vi "Create Message Accessor.vi"(8 "error in (no error)":errorcluster, 10 "message name":string, 11 "library in":refnum<vi>) -> (0 "error out":errorcluster, 3 "library out":refnum<vi>)   [LabVIEW 2019, in "gRPC Template Creation Utility.lvlib"]
uses:
  gRPC Template Creation Utility.lvlib
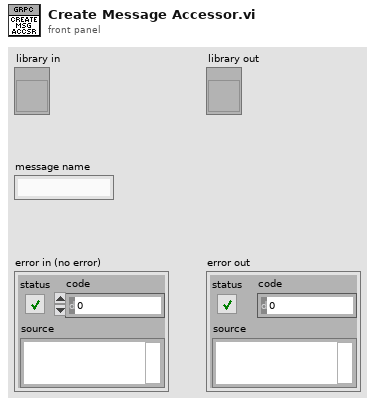
[diagram p1: front panel]
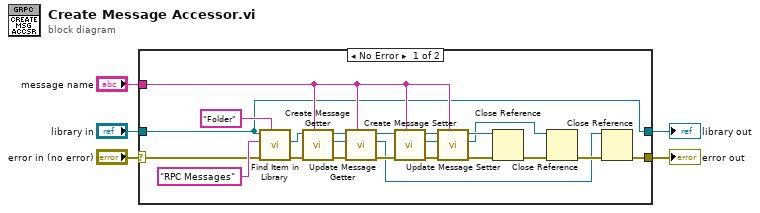
[diagram p0: block diagram]
diagram:
  n1 = case shown="No Error" "error in (no error)" {
    selector: "error in (no error)" -> [w15 w28]
    tunnel: "library in" -> [w14 w29]
    tunnel: "message name" -> [w27 _]
    tunnel: [w16 w28] -> w4
    tunnel: [w14 w29] -> w2
    frame No Error {
      n2 = call "Find Item in Library.vi"("Item Type"="Folder", "error in (no error)"=w15, "Item Name"="RPC Messages", "Library item in"=w14) -> ("error out"=w13:errorcluster, "Project Item (Library Item)"=w21:refnum<vi>)  [unwired: 4 in, 2 out]
      n3 = call "Create Message Getter.vi"("RPC Message Name"=w27, "error in (no error)"=w13, "RPC Messages Folder (ProjectItem) in"=w21) -> ("error out"=w22:errorcluster, "Message Getter out"=w23:refnum<vi>, "RPC Messages Folder (ProjectItem) out"=w24:refnum<vi>)  [unwired: 6 in]
      n4 = call "Update Message Getter.vi"("RPC Message Name"=w27, "error in (no error)"=w22, "Message Getter in"=w23, "RPC Messages Folder (ProjectItem) in"=w24) -> ("error out"=w12:errorcluster, "Message Getter out"=w7:refnum<vi>, "RPC Messages Folder (ProjectItem) out"=w11:refnum<vi>)  [unwired: 5 in]
      n5 = call "Create Message Setter.vi"("RPC Message Name"=w27, "error in (no error)"=w12, "RPC Messages Folder (ProjectItem) in"=w11) -> ("error out"=w20:errorcluster, "Message Setter out"=w18:refnum<vi>, "RPC Messages Folder (ProjectItem) out"=w19:refnum<vi>)  [unwired: 6 in]
      n6 = call "Update Message Setter.vi"("RPC Message Name"=w27, "error in (no error)"=w20, "Message Getter in"=w18, "RPC Messages Folder (ProjectItem) in"=w19) -> ("error out"=w17:errorcluster, "Message Getter out"=w6:refnum<vi>, "RPC Messages Folder (ProjectItem) out"=w8:refnum<vi>)  [unwired: 5 in]
      n7 = Close Reference(reference=w8, error in (no error)=w17) -> (error out=w10:errorcluster)
      n8 = Close Reference(reference=w6, error in (no error)=w10) -> (error out=w9:errorcluster)
      n9 = Close Reference(reference=w7, error in (no error)=w9) -> (error out=w16:errorcluster)
    }
    frame Error {
    }
  }
  "error out" <- w4
  "library out" <- w2
